vi "Merge Image - Transform and Cast to U8.vi"(0 "Selected Image (U8 or U16)":T2[](array[typedef]), 1 "Dummy Image Ref":T2, 3 "Transform Parameters":T1[](array[typedef]) {"Image" items=["None"]}, 7 "RGB Image Refs (U8)":T2[](array[typedef]), 11 "RGB Image Refs (U16)":T2[](array[typedef]), 13 "Image Holds":bool[](array[boolean])=[FALSE, FALSE, FALSE]) -> (8 "RGB Image Refs (U8 DUP)":T2[](array[typedef]))   [LabVIEW 2016]
uses:
  <vilib>/vision/Image Controls.llb/IMAQ Image.ctl
  Merge Image Type Defs/Merge Image - Image Control.ctl
  <vilib>/vision/NI_Vision_Development_Module.lvlib
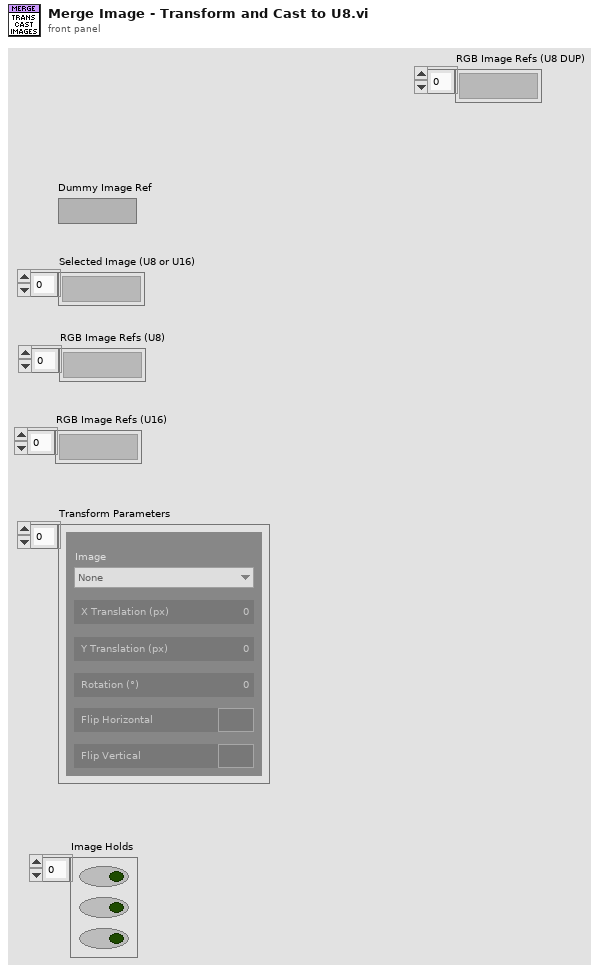
[diagram p1: front panel]
types:
  T1 = typedef "Merge Image - Image Control.ctl" = cluster{"Image":i32, "X Translation (px)":i32, "Y Translation (px)":i32, "Rotation (°)":sgl, "Flip Horizontal":bool, "Flip Vertical":bool}
  T2 = typedef "IMAQ Image.ctl" = refnum<image>
  T3 = typedef "Image Type" = u32
  T4 = cluster{"Mean Value":sgl, "Standard Variation":sgl, "Minimal Value":sgl, "Maximal Value":sgl, "Area (calibrated)":sgl, "Area (pixels)":u32, "%":sgl, "Calibration Valid":bool}
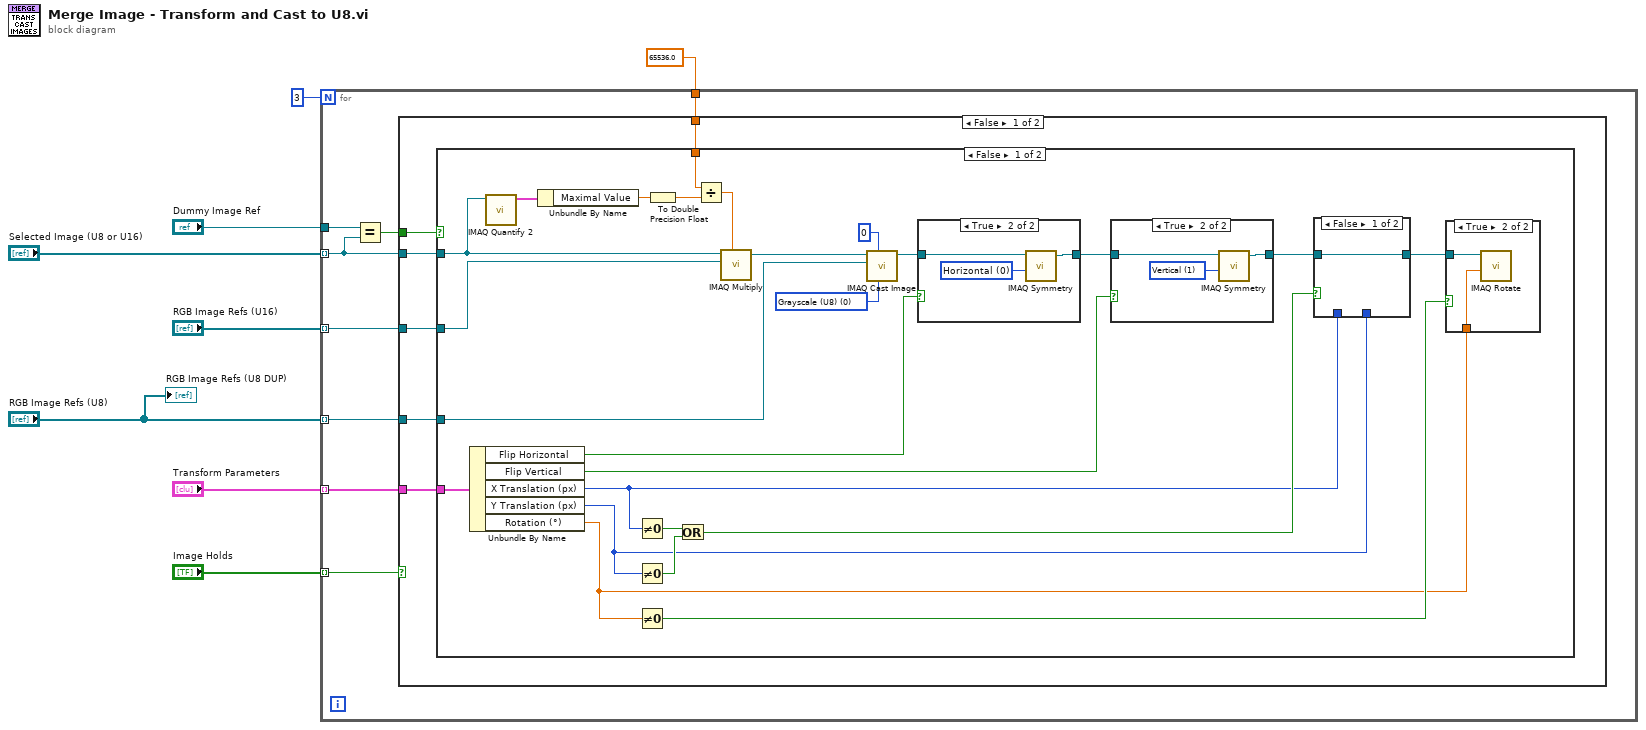
[diagram p0: block diagram]
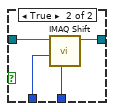
[diagram p3: hidden frame]
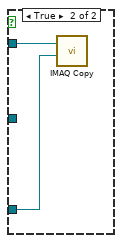
[diagram p6: hidden frame]
diagram:
  n1 = for {
    N: 3 -> [_]
    tunnel: "Selected Image (U8 or U16)" -> [w13] mode=indexing
    tunnel: "Dummy Image Ref" -> [w16]
    tunnel: "RGB Image Refs (U8)" -> [w14] mode=indexing
    tunnel: 65536.0 -> [w12]
    tunnel: "RGB Image Refs (U16)" -> [w11] mode=indexing
    tunnel: "Transform Parameters" -> [w10] mode=indexing
    tunnel: "Image Holds" -> [w9] mode=indexing
    n2 = Equal?(x=w16, y=w13) -> (x = y?=w15:bool)
    n3 = case shown="False" w9 {
      tunnel: w15 -> [w22 _]
      tunnel: w14 -> [w21 _]
      tunnel: w13 -> [w20 _]
      tunnel: w12 -> [w19 _]
      tunnel: w11 -> [w18 _]
      tunnel: w10 -> [w17 _]
      frame False {
        n4 = case shown="False" w22 {
          tunnel: w21 -> [w39 w63]
          tunnel: w20 -> [w43 w64]
          tunnel: w19 -> [w44 _]
          tunnel: w18 -> [w41 _]
          tunnel: w17 -> [w36 _]
          frame False {
            w37 = T3 0 items=["Grayscale (U8)", "Grayscale (I16)", "Grayscale (SGL)", "Complex (CSG)", "RGB (U32)", "HSL (U32)", "RGB (U64)", "Grayscale (U16)"] ("Image Type")
            n5 = Unbundle By Name(w36) -> ("Flip Horizontal"=w34:bool, "Flip Vertical"=w32:bool, "X Translation (px)"=w27:i32, "Y Translation (px)"=w26:i32, "Rotation (°)"=w23:sgl)
            n6 = call "IMAQ Quantify 2"("Image"=w43) -> ("Global Report"=w45:T4)  [unwired: 8 in, 2 out]
            n7 = Unbundle By Name(w45) -> ("Maximal Value"=w46:sgl)
            n8 = Not Equal To 0?(x=w27) -> (x != 0?=w31:bool)
            n9 = Not Equal To 0?(x=w26) -> (x != 0?=w30:bool)
            n10 = Not Equal To 0?(x=w23) -> (x != 0?=w25:bool)
            n11 = To Double Precision Float(number=w46) -> (double precision float=w47:dbl)
            n12 = Or(x=w31, y=w30) -> (x .or. y?=w29:bool)
            n13 = Divide(x=w44, y=w47) -> (x/y=w42:dbl)
            n14 = call "IMAQ Multiply"("Image Src A"=w43, "Constant"=w42, "Image Dst"=w41) -> ("Image Dst Out"=w40:T2)  [unwired: 4 in, 1 out]
            n15 = call "IMAQ Cast Image"("Image Type"=w37, "# Shifts"=0, "Image Dst"=w39, "Image Src"=w40) -> ("Image Dst Out"=w35:T2)  [unwired: 6 in, 1 out]
            n16 = case shown="True" w34 {
              tunnel: w35 -> [w59 w62]
              tunnel: [w59 w60] -> w33
              frame False {
              }
              frame True {
                w61 = u32 0 items=["Horizontal", "Vertical", "Central", "1st Diagonal", "2nd Diagonal"] ("Type of Symmetry")
                n17 = call "IMAQ Symmetry"("Type of Symmetry"=w61, "Image Src"=w62) -> ("Image Dst Out"=w60:T2)  [unwired: 3 in, 1 out]
              }
            }
            n18 = case shown="True" w32 {
              tunnel: w33 -> [w55 w58]
              tunnel: [w55 w56] -> w28
              frame False {
              }
              frame True {
                w57 = u32 1 items=["Horizontal", "Vertical", "Central", "1st Diagonal", "2nd Diagonal"] ("Type of Symmetry")
                n19 = call "IMAQ Symmetry"("Type of Symmetry"=w57, "Image Src"=w58) -> ("Image Dst Out"=w56:T2)  [unwired: 3 in, 1 out]
              }
            }
            n20 = case shown="False" w29 {
              tunnel: w28 -> [w50 w54]
              tunnel: w27 -> [_ w53]
              tunnel: w26 -> [_ w52]
              tunnel: [w50 w51] -> w24
              frame False {
              }
              frame True {
                n21 = call "IMAQ Shift"("YOffset"=w52, "XOffset"=w53, "Image Src"=w54) -> ("Image Dst Out"=w51:T2)  [unwired: 7 in, 1 out]
              }
            }
            n22 = case shown="True" w25 {
              tunnel: w24 -> [_ w49]
              tunnel: w23 -> [_ w48]
              frame False {
              }
              frame True {
                n23 = call "IMAQ Rotate"("Angle (degrees)"=w48, "Image Src"=w49) -> ()  [unwired: 8 in, 2 out]
              }
            }
          }
          frame True {
            n24 = call "IMAQ Copy"("Image Dst"=w63, "Image Src"=w64) -> ()  [unwired: 4 in, 2 out]
          }
        }
      }
      frame True {
      }
    }
  }
  "RGB Image Refs (U8 DUP)" <- "RGB Image Refs (U8)"
